vi "PAQmem_ReadArray.vi"(8 "error in (no error)":errorcluster, 10 "ChunkDefinition":T2, 11 "PAQ-memory in":refnum<class "PAQ-memory.lvclass">) -> (0 "error out":errorcluster, 2 "OneTagData":T1, 3 "PAQ-memory out":refnum<class "PAQ-memory.lvclass">)   [LabVIEW 2020, in "Sgraph_lib_V1.lvlib" / "PAQ-memory.lvclass"]
doc: "For One TAG get an Array of data"
uses:
  PAQ-memory.lvclass
  PAQ-memory.lvclass/PAQ-memory.ctl
  <vilib>/Utility/error.llb/Error Cluster From Error Code.vi
  <vilib>/ErrorRing/Error Ring.xnode
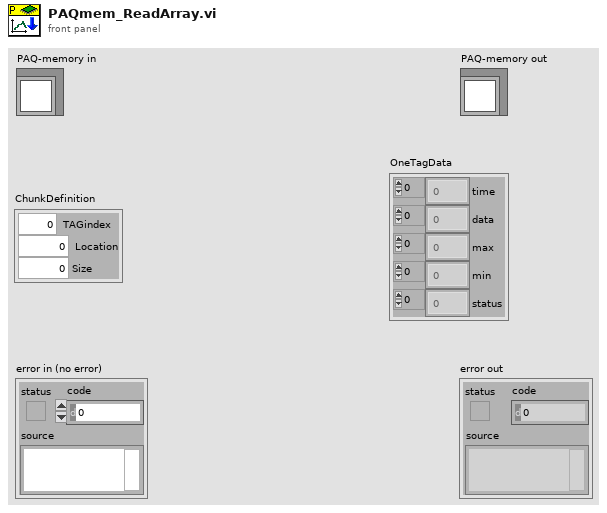
[diagram p1: front panel]
types:
  T1 = cluster{"time":dbl[], "data":dbl[], "max":dbl[], "min":dbl[], "status":u32[]}
  T2 = cluster{"TAGindex":i32, "Location":i32, "Size":i32}
  T3 = cluster{"source":refnum<data-value>, "status":refnum<data-value>, "data":refnum<data-value>, "max":refnum<data-value>, "min":refnum<data-value>}[]
  T4 = cluster{"source":refnum<data-value>, "status":refnum<data-value>, "data":refnum<data-value>, "max":refnum<data-value>, "min":refnum<data-value>}
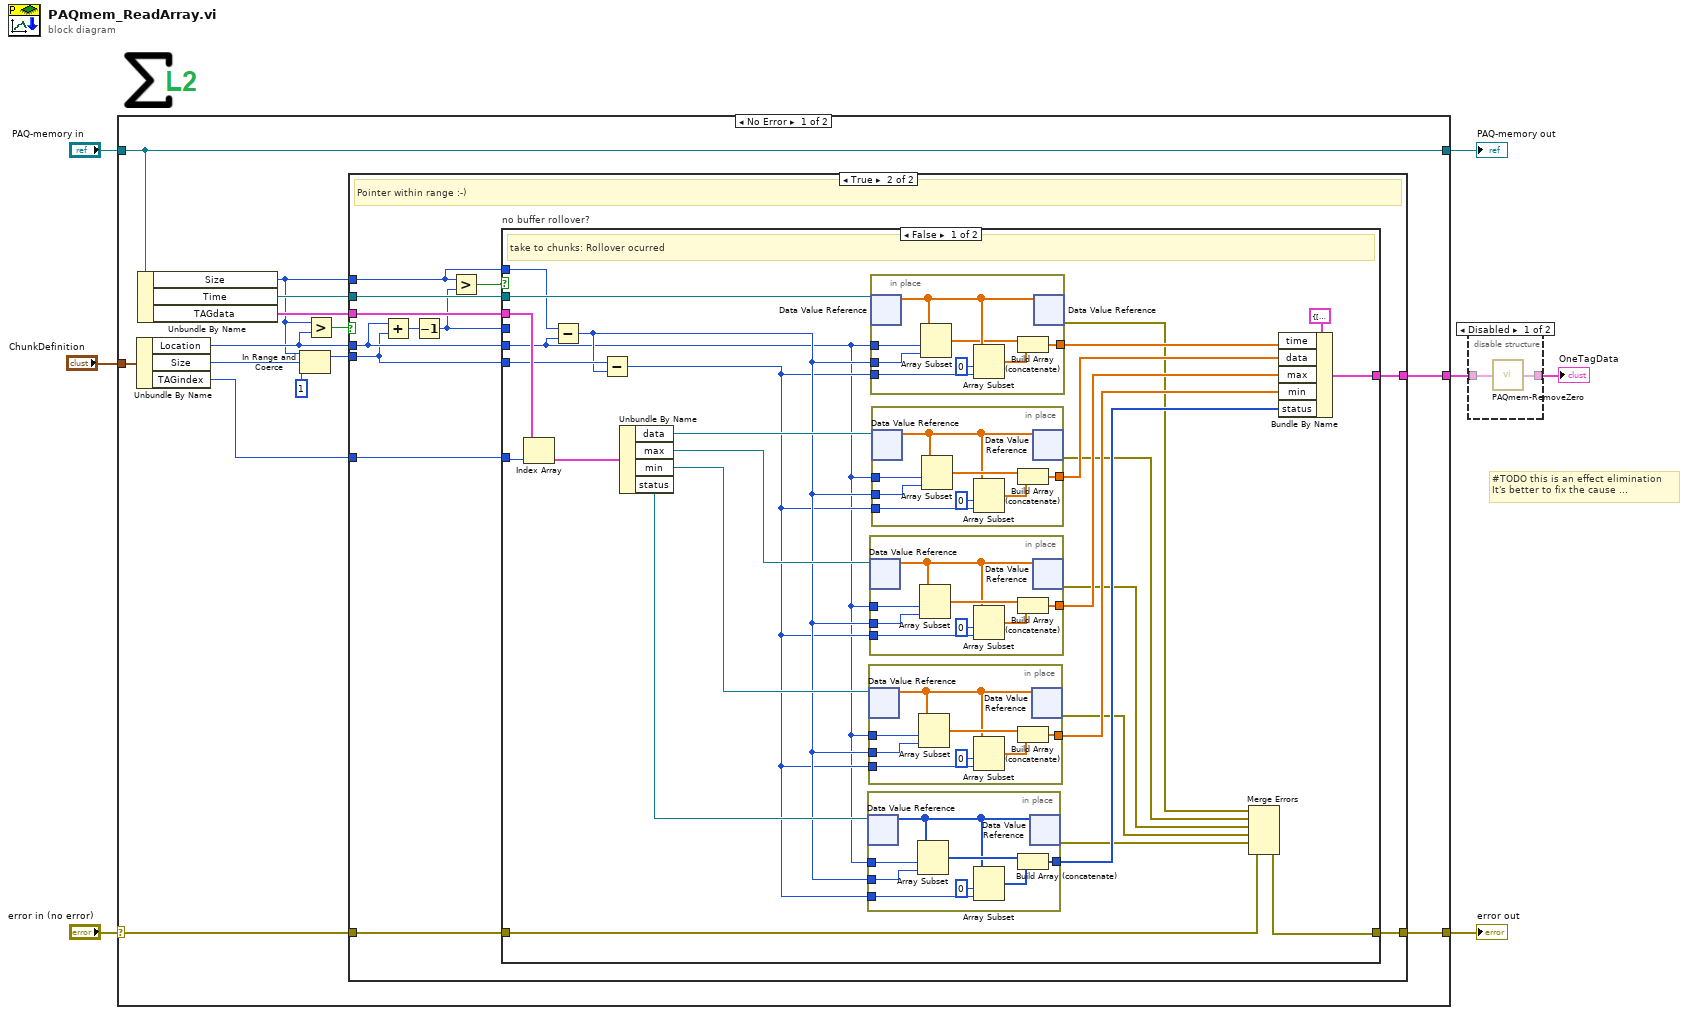
[diagram p0: block diagram]
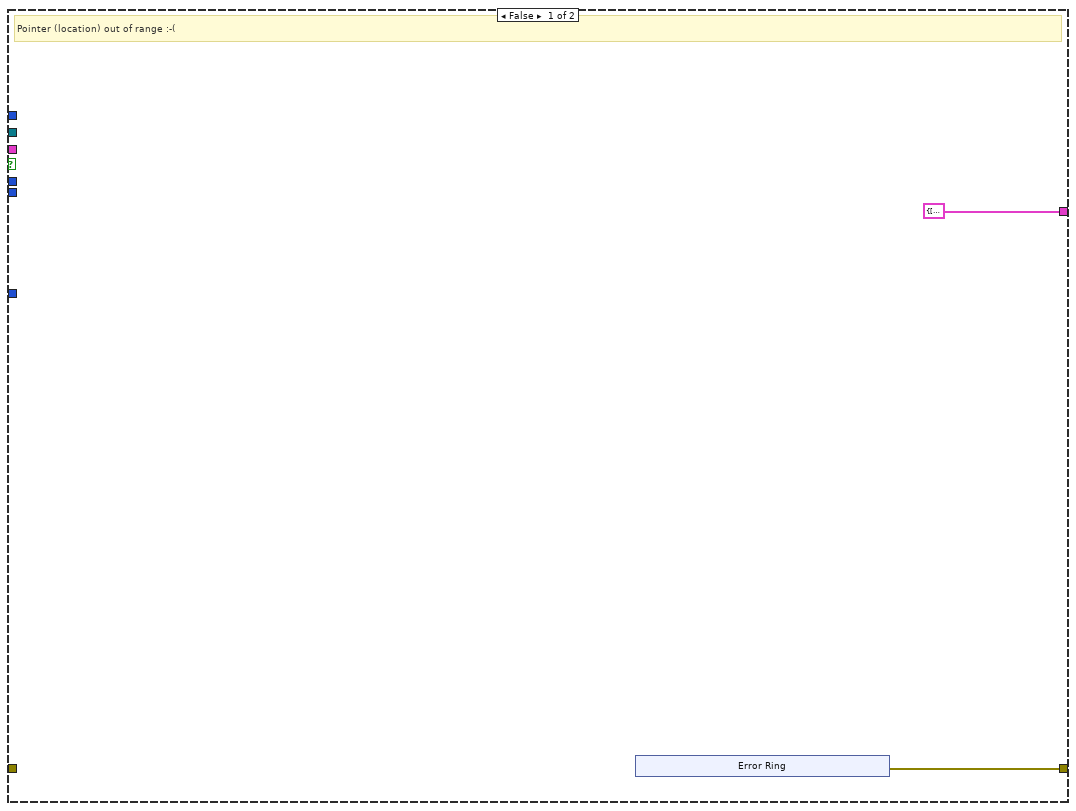
[diagram p3: hidden frame]
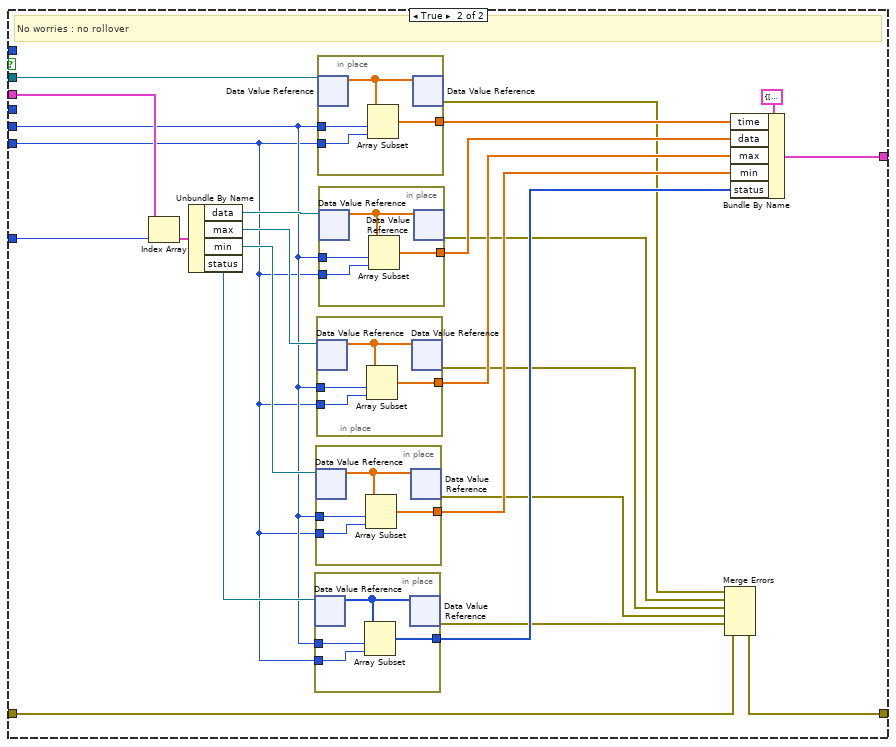
[diagram p4: hidden frame]
diagram:
  # "#TODO this is an effect elimination\nIt's better to fix the cause ..."
  n1 = case shown="No Error" "error in (no error)" {
    selector: "error in (no error)" -> [w15 w153]
    tunnel: [w14 w153] -> w6
    tunnel: [w20 w152] -> w4
    tunnel: "PAQ-memory in" -> [w20 w152]
    tunnel: "ChunkDefinition" -> [w21 _]
    tunnel: [w18 _] -> w2
    frame No Error {
      n2 = Unbundle By Name(w21) -> ("Location"=w13:i32, "Size"=w10:i32, "TAGindex"=w16:i32)
      n3 = Unbundle By Name(w20) -> ("Size"=w11:i32, "Time"=w19:refnum<data-value>, "TAGdata"=w17:T3)
      n4 = In Range and Coerce(upper limit=w11, x=w10, lower limit=1) -> (coerced(x)=w9:i32)  [unwired: 1 out]
      n5 = Greater?(x=w11, y=w13) -> (0:w12:bool)
      n6 = case shown="True" w12 {
        tunnel: w19 -> [_ w40]
        tunnel: [T1 {"time"=[], "data"=[], "max"=[], "min"=[], "status"=[]} ("GraphData") w39] -> w18
        tunnel: w17 -> [_ w38]
        tunnel: w16 -> [_ w37]
        tunnel: w9 -> [_ w33]
        tunnel: w15 -> [_ w36]
        tunnel: [w22 w35] -> w14
        tunnel: w13 -> [_ w34]
        tunnel: w11 -> [_ w30]
        frame False {
          # "Pointer (location) out of range :-("
          n7 = xnode "Error Ring"() -> ("error out"=w22:errorcluster)
        }
        frame True {
          # "Pointer within range :-)"
          n8 = Add(x=w34, y=w33) -> (x+y=w32:i32)
          n9 = Decrement(x=w32) -> (x-1=w29:i32)
          n10 = Greater?(x=w30, y=w29) -> (0:w31:bool)
          n11 = case "no buffer rollover?" shown="False" w31 {
            tunnel: w40 -> [w63 w131]
            tunnel: [w55 w129] -> w39
            tunnel: w38 -> [w62 w127]
            tunnel: w37 -> [w61 w126]
            tunnel: w36 -> [w49 w116]
            tunnel: [w43 w110] -> w35
            tunnel: w34 -> [w41 w109]
            tunnel: w33 -> [w59 w108]
            tunnel: w30 -> [w42 _]
            tunnel: w29 -> [_ _]
            frame False {
              # "take to chunks: Rollover ocurred"
              n12 = Index Array(array=w62, index=w61) -> (element=w60:T4)
              n13 = Subtract(x=w42, y=w41) -> (x-y=w58:i32)
              n14 = Subtract(x=w59, y=w58) -> (x-y=w57:i32)
              n15 = Unbundle By Name(w60) -> ("data"=w64:refnum<data-value>, "max"=w65:refnum<data-value>, "min"=w66:refnum<data-value>, "status"=w67:refnum<data-value>)
              n16 = in-place {
                in-place-border: w41 -> [w75]
                in-place-border: w58 -> [w74]
                in-place-border: w57 -> [w72]
                in-place-border: [w68] -> w50
                n17 = in-place-dvr #1(w67) -> (w69:u32[])  [unwired: 1 out]
                n18 = Array Subset(array=w69, index=w75, length=w74) -> (w71:u32[])
                n19 = Array Subset(array=w69, index=0, length=w72) -> (w70:u32[])
                n20 = Build Array (concatenate)(w71, w70) -> (w68:u32[])
                n21 = in-place-dvr #1(w69) -> (w48:errorcluster)  [unwired: 1 out]
              }
              n22 = in-place {
                in-place-border: w41 -> [w83]
                in-place-border: w58 -> [w82]
                in-place-border: w57 -> [w80]
                in-place-border: [w76] -> w51
                n23 = in-place-dvr #2(w66) -> (w77:dbl[])  [unwired: 1 out]
                n24 = Array Subset(array=w77, index=w83, length=w82) -> (w79:dbl[])
                n25 = Array Subset(array=w77, index=0, length=w80) -> (w78:dbl[])
                n26 = Build Array (concatenate)(w79, w78) -> (w76:dbl[])
                n27 = in-place-dvr #2(w77) -> (w47:errorcluster)  [unwired: 1 out]
              }
              n28 = in-place {
                in-place-border: w41 -> [w91]
                in-place-border: w58 -> [w90]
                in-place-border: w57 -> [w88]
                in-place-border: [w84] -> w52
                n29 = in-place-dvr #3(w65) -> (w85:dbl[])  [unwired: 1 out]
                n30 = Array Subset(array=w85, index=w91, length=w90) -> (w87:dbl[])
                n31 = Array Subset(array=w85, index=0, length=w88) -> (w86:dbl[])
                n32 = Build Array (concatenate)(w87, w86) -> (w84:dbl[])
                n33 = in-place-dvr #3(w85) -> (w46:errorcluster)  [unwired: 1 out]
              }
              n34 = in-place {
                in-place-border: w41 -> [w107]
                in-place-border: w58 -> [w106]
                in-place-border: w57 -> [w103]
                in-place-border: [w100] -> w54
                n35 = in-place-dvr #4(w63) -> (w104:dbl[])  [unwired: 1 out]
                n36 = Array Subset(array=w104, index=w107, length=w106) -> (w102:dbl[])
                n37 = Array Subset(array=w104, index=0, length=w103) -> (w101:dbl[])
                n38 = Build Array (concatenate)(w102, w101) -> (w100:dbl[])
                n39 = in-place-dvr #4(w104) -> (w44:errorcluster)  [unwired: 1 out]
              }
              n40 = in-place {
                in-place-border: w41 -> [w99]
                in-place-border: w58 -> [w98]
                in-place-border: w57 -> [w96]
                in-place-border: [w92] -> w53
                n41 = in-place-dvr #5(w64) -> (w93:dbl[])  [unwired: 1 out]
                n42 = Array Subset(array=w93, index=w99, length=w98) -> (w95:dbl[])
                n43 = Array Subset(array=w93, index=0, length=w96) -> (w94:dbl[])
                n44 = Build Array (concatenate)(w95, w94) -> (w92:dbl[])
                n45 = in-place-dvr #5(w93) -> (w45:errorcluster)  [unwired: 1 out]
              }
              n46 = Merge Errors(w44, w45, w46, w47, w48, w49) -> (w43:errorcluster)
              n47 = Bundle By Name(cluster=T1 {"time"=[], "data"=[], "max"=[], "min"=[], "status"=[]} ("GraphData"), "time"=w54, "data"=w53, "max"=w52, "min"=w51, "status"=w50) -> (w55:T1)
            }
            frame True {
              # "No worries : no rollover"
              n48 = Index Array(array=w127, index=w126) -> (element=w125:T4)
              n49 = Unbundle By Name(w125) -> ("data"=w124:refnum<data-value>, "max"=w123:refnum<data-value>, "min"=w122:refnum<data-value>, "status"=w121:refnum<data-value>)
              n50 = in-place {
                in-place-border: w109 -> [w134]
                in-place-border: w108 -> [w133]
                in-place-border: [w132] -> w117
                n51 = in-place-dvr #6(w121) -> (w135:u32[])  [unwired: 1 out]
                n52 = Array Subset(array=w135, index=w134, length=w133) -> (w132:u32[])
                n53 = in-place-dvr #6(w135) -> (w115:errorcluster)  [unwired: 1 out]
              }
              n54 = in-place {
                in-place-border: w109 -> [w138]
                in-place-border: w108 -> [w137]
                in-place-border: [w136] -> w118
                n55 = in-place-dvr #7(w122) -> (w139:dbl[])  [unwired: 1 out]
                n56 = Array Subset(array=w139, index=w138, length=w137) -> (w136:dbl[])
                n57 = in-place-dvr #7(w139) -> (w114:errorcluster)  [unwired: 1 out]
              }
              n58 = in-place {
                in-place-border: w109 -> [w142]
                in-place-border: w108 -> [w141]
                in-place-border: [w140] -> w119
                n59 = in-place-dvr #8(w123) -> (w143:dbl[])  [unwired: 1 out]
                n60 = Array Subset(array=w143, index=w142, length=w141) -> (w140:dbl[])
                n61 = in-place-dvr #8(w143) -> (w113:errorcluster)  [unwired: 1 out]
              }
              n62 = in-place {
                in-place-border: w109 -> [w150]
                in-place-border: w108 -> [w149]
                in-place-border: [w148] -> w128
                n63 = in-place-dvr #9(w131) -> (w151:dbl[])  [unwired: 1 out]
                n64 = Array Subset(array=w151, index=w150, length=w149) -> (w148:dbl[])
                n65 = in-place-dvr #9(w151) -> (w111:errorcluster)  [unwired: 1 out]
              }
              n66 = in-place {
                in-place-border: w109 -> [w146]
                in-place-border: w108 -> [w145]
                in-place-border: [w144] -> w120
                n67 = in-place-dvr #10(w124) -> (w147:dbl[])  [unwired: 1 out]
                n68 = Array Subset(array=w147, index=w146, length=w145) -> (w144:dbl[])
                n69 = in-place-dvr #10(w147) -> (w112:errorcluster)  [unwired: 1 out]
              }
              n70 = Merge Errors(w111, w112, w113, w114, w115, w116) -> (w110:errorcluster)
              n71 = Bundle By Name(cluster=T1 {"time"=[], "data"=[], "max"=[], "min"=[], "status"=[]} ("GraphData"), "time"=w128, "data"=w120, "max"=w119, "min"=w118, "status"=w117) -> (w129:T1)
            }
          }
        }
      }
    }
    frame Error {
    }
  }
  "error out" <- w6
  "PAQ-memory out" <- w4
  n72 = disable-structure shown="Disabled" {
    disable-tunnel: w2 -> [w155 w156]
    disable-tunnel: [w154 w156] -> w1
    frame Disabled {
      n73 = call "PAQmem-RemoveZero.vi"("OneTagData in"=w155) -> ("OneTagData out"=w154:T1)  [unwired: 8 in]
    }
    frame Enabled {
    }
  }
  "OneTagData" <- w1
